vi "RDV-writeIgnoreList.vi"(8 "error in (no error)":errorcluster, 10 "Keys to ignore":T1, 11 "RDV-Reflection_Data_viewer in":refnum<class "RDV-Reflection_Data_viewer.lvclass">) -> (0 "error out":errorcluster, 3 "RDV-Reflection_Data_viewer out":refnum<class "RDV-Reflection_Data_viewer.lvclass">)   [LabVIEW 2020, in "RDV-Reflection_Data_viewer.lvclass"]
doc: "Writes the list of keys to ignore into the viewer object."
uses:
  RDV-Reflection_Data_viewer.lvclass
  RDV-UPDATE_IGNORE_LIST.ctl
  RDV-Reflection_Data_viewer.lvclass/RDV-Reflection_Data_viewer.ctl
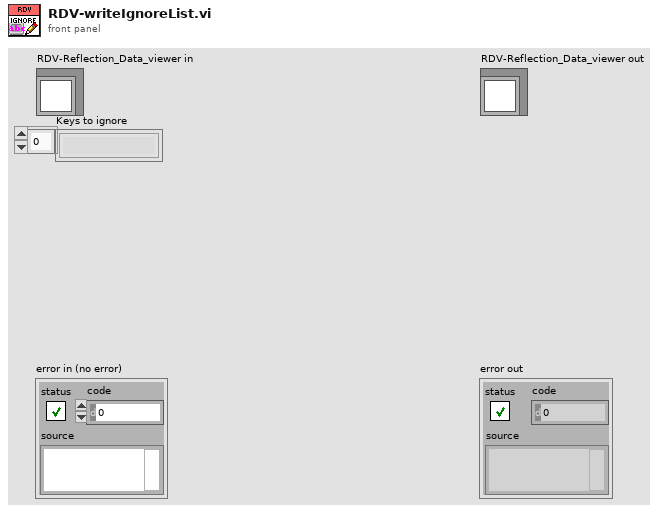
[diagram p1: front panel]
types:
  T1 = typedef "RDV-Reflection_Data_viewer.lvclass/RDV-UPDATE_IGNORE_LIST.ctl" = string[]
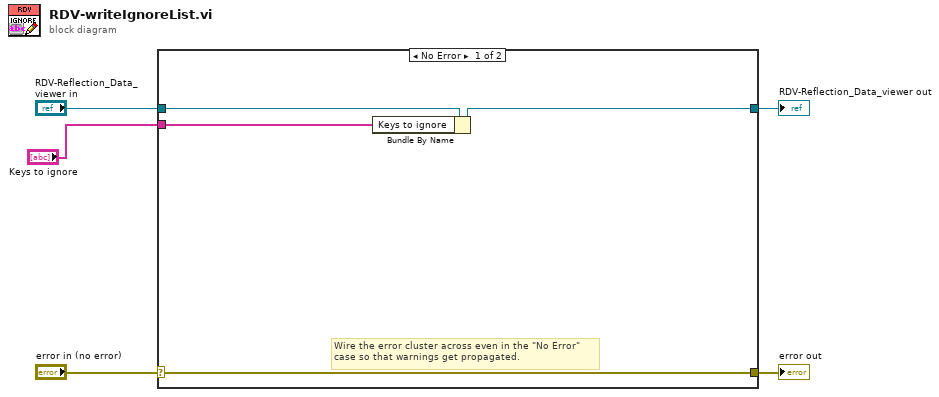
[diagram p0: block diagram]
diagram:
  n1 = case shown="No Error" "error in (no error)" {
    selector: "error in (no error)" -> [w8 w11]
    tunnel: [w8 w11] -> w4
    tunnel: [w7 w10] -> w2
    tunnel: "RDV-Reflection_Data_viewer in" -> [w9 w10]
    tunnel: "Keys to ignore" -> [w6 _]
    frame No Error {
      # "Wire the error cluster across even in the \"No Error\"\ncase so that warnings get propagated."
      n2 = Bundle By Name(cluster=w9, "Keys to ignore"=w6) -> (w7:refnum<class "RDV-Reflection_Data_viewer.lvclass">)
    }
    frame Error {
    }
  }
  "error out" <- w4
  "RDV-Reflection_Data_viewer out" <- w2
